vi "real-time OS check.vi"(8 "error in":errorcluster, 11 "system session":refnum<k21>) -> (0 "error out":errorcluster, 3 "system session out":refnum<k21>)   [LabVIEW 2014, in "SMI.lvlib" / "SysCfg Device.lvclass"]
uses:
  SysCfg Device.lvclass
  <resource>/objmgr/nisysapi.rc
  SMI.lvlib
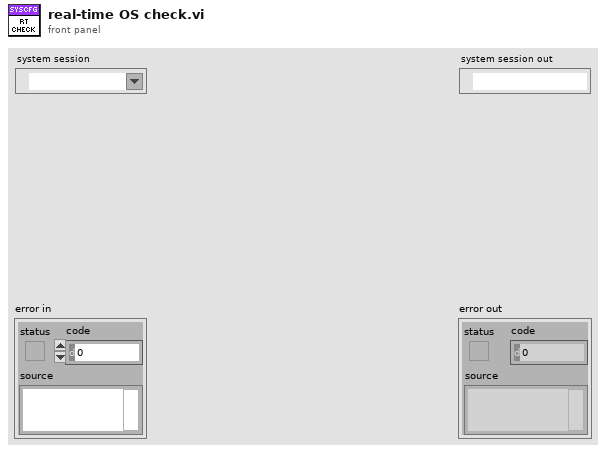
[diagram p1: front panel]
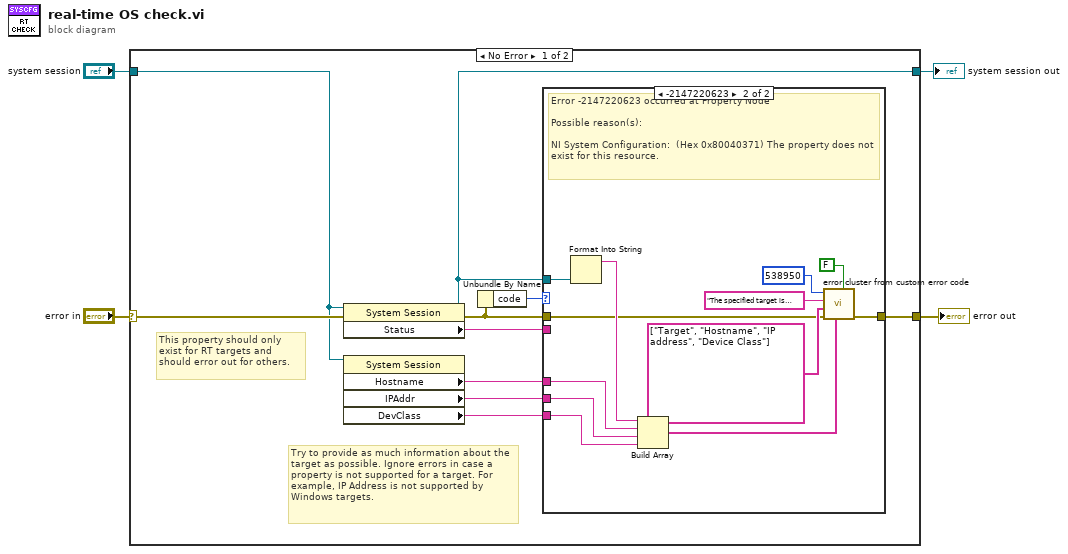
[diagram p0: block diagram]
diagram:
  n1 = case shown="No Error" "error in" {
    selector: "error in" -> [w14 w29]
    tunnel: [w11 w29] -> w2
    tunnel: "system session" -> [w8 w28]
    tunnel: [w9 w28] -> w4
    frame No Error {
      # "Try to provide as much information about the target as possible. Ignore errors in case a property is not supported for a target. For example, IP Address is not supported by Windows targets."
      # "This property should only exist for RT targets and should error out for others."
      n2 = property class="System Session"(reference=w8, error in=w14) -> (reference out=w9:refnum<k21>, error out=w12:errorcluster, "Status"=w10:string)
      n3 = property class="System Session"(reference=w8) -> ("Hostname"=w7:string, "IPAddr"=w6:string, "DevClass"=w5:string)  [unwired: 1 in, 2 out]
      n4 = Unbundle By Name(w12) -> ("code"=w13:i32)
      n5 = case shown="-2147220623" w13 {
        tunnel: w12 -> [w15 w16]
        tunnel: [w15 w27] -> w11
        tunnel: w10 -> [_ _]
        tunnel: w9 -> [_ w26]
        tunnel: w7 -> [_ w19]
        tunnel: w6 -> [_ w18]
        tunnel: w5 -> [_ w17]
        frame Default {
        }
        frame -2147220623 {
          # "Error -2147220623 occurred at Property Node\n\nPossible reason(s):\n\nNI System Configuration:  (Hex 0x80040371) The property does not exist for this resource."
          n6 = Format Into String(w26) -> (resulting string=w20:string)  [unwired: 3 in, 1 out]
          n7 = Build Array(w20, w19, w18, w17) -> (w23:string[])
          n8 = call "error cluster from custom error code.vi"("is warning? (True)"=FALSE, "string values"=w23, "error in"=w16, "keys"=string[] ["Target", "Hostname", "IP address", "Device Class"], "error message"="The specified target is unsupported. SMI is only intended for real-time targets.", "custom error code (0)"=538950 ("error code (0)")) -> ("error out"=w27:errorcluster)  [unwired: 5 in]
        }
      }
    }
    frame Error {
    }
  }
  "error out" <- w2
  "system session out" <- w4
